vi "MQTT Data Stream - Decode HEADER.vi"(0 "TCP ref":refnum<k5>, 9 "timeout ms (1000)":i32, 11 "error in (no error)":errorcluster) -> (3 "RAW Data":string, 4 "TCP ref out":refnum<k5>, 6 "Fixed Header":T1, 15 "error out":errorcluster)   [LabVIEW 2019, in "KoRE-MQTT.lvlib"]
doc: "Decodes the MQTT fixed header byte.\n\n\nCopyright (c) 2025 KoRElibs.com\nSPDX-License-Identifier: EUPL-1.2\n\nThis VI is licensed under the European Union Public License (EUPL) Version 1.2. You may use this VI unmodified in proprietary works. If you distribute a modified version of this file, the modified file must be released under the EUPL-1.2. Full license: https://joinup.ec.europa.eu/asset/eupl/eupl/1.2/"
uses:
  KoRE-MQTT.lvlib
  TypeDefs/MQTT Packet - Fixed Header.ctl
  TypeDefs/MQTT Packet - Type.ctl
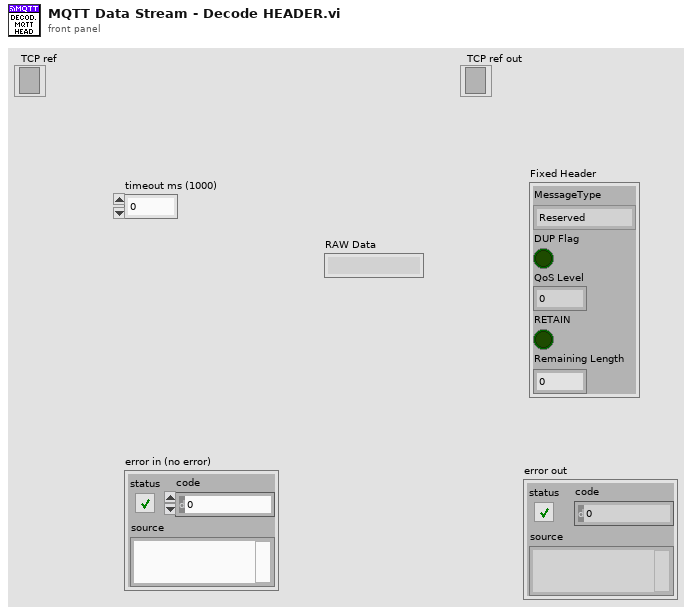
[diagram p1: front panel]
types:
  T1 = typedef "KoRE-MQTT.lvlib/MQTT Packet - Fixed Header.ctl" = cluster{"MessageType":T2, "DUP Flag":bool, "QoS Level":u8, "RETAIN":bool, "Remaining Length":u32}
  T2 = typedef "KoRE-MQTT.lvlib/MQTT Packet - Type.ctl" = enum32{"Reserved", "CONNECT", "CONNACK", "PUBLISH", "PUBACK", "PUBREC", "PUBREL", "PUBCOMP", "SUBSCRIBE", "SUBACK", "UNSUBSCRIBE", "UNSUBACK", "PINGREQ", "PINGRESP", "DISCONNECT", "AUTH"}
  T3 = enum16{"Standard", "Buffered", "CRLF", "Immediate"}
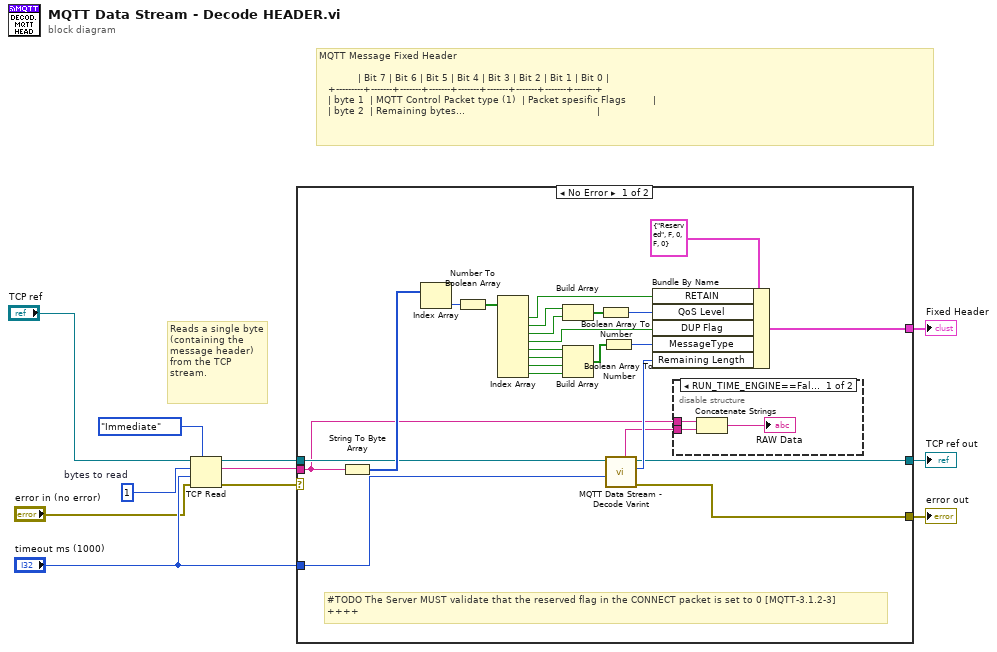
[diagram p0: block diagram]
diagram:
  w6 = 1  # bytes to read
  # "MQTT Message Fixed Header\n\n             | Bit 7 | Bit 6 | Bit 5 | Bit 4 | Bit 3 | Bit 2 | Bit 1 | Bit 0 |\n   +---------+-------+-------+-------+-------+-------+-------+-------+-------+\n   | byte 1  | MQTT Control Packet type (1)  | Packet spesific Flags         |\n   | byte 2  | Remaining bytes...                                            |"
  # "Reads a single byte (containing the message header) from the TCP stream."
  n1 = TCP Read(connection ID="TCP ref", bytes to read=w6, error in (no error)="error in (no error)", 7:T3."Immediate" ("mode (standard)"), 9:"timeout ms (1000)") -> (connection ID out=w7:refnum<k5>, data out=w9:string, error out=w4:errorcluster)
  n2 = case shown="No Error" w4 {
    selector: w4 -> [_ w40]
    tunnel: [w35 _] -> w11
    tunnel: "timeout ms (1000)" -> [w19 _]
    tunnel: w9 -> [w14 _]
    tunnel: w7 -> [w18 w39]
    tunnel: [w17 w40] -> w5
    tunnel: [w12 w39] -> w1
    frame No Error {
      # "#TODO The Server MUST validate that the reserved flag in the CONNECT packet is set to 0 [MQTT-3.1.2-3]\n++++"
      n3 = String To Byte Array(string=w14) -> (unsigned byte array=w31:u8[])
      n4 = Index Array(array=w31) -> (element=w20:u8)  [unwired: 1 in]
      n5 = Number To Boolean Array(number=w20) -> (Boolean array=w21:bool[])
      n6 = Index Array(array=w21) -> (element #1=w33:bool, element #2=w22:bool, element #3=w23:bool, element #4=w34:bool, element #5=w25:bool, element #6=w26:bool, element #7=w27:bool, element #8=w28:bool)  [unwired: 8 in]
      n7 = Build Array(w22, w23) -> (w24:bool[])
      n8 = Build Array(w25, w26, w27, w28) -> (w29:bool[])
      n9 = Boolean Array To Number(Boolean array=w24) -> (number=w15:u32)
      n10 = Boolean Array To Number(Boolean array=w29) -> (number=w16:u32)
      n11 = call "MQTT Data Stream - Decode Varint.vi"("timeout ms (1000)"=w19, "TCP Network Connection in"=w18) -> ("error out"=w17:errorcluster, "Numeric"=w32:u32, "TCP Network Connection out"=w12:refnum<k5>, "RAW data"=w13:string)  [unwired: 5 in, 1 out]
      n12 = Bundle By Name(cluster=T1 {"MessageType"=enum."Reserved", "DUP Flag"=FALSE, "QoS Level"=0, "RETAIN"=FALSE, "Remaining Length"=0} ("Fixed Header"), "RETAIN"=w33, "QoS Level"=w15, "DUP Flag"=w34, "MessageType"=w16, "Remaining Length"=w32) -> (w35:T1)
      n13 = disable-structure shown="RUN_TIME_ENGINE==False" {
        disable-tunnel: w14 -> [w38 _]
        disable-tunnel: w13 -> [w37 _]
        frame condition #0 (active) {
          n14 = Concatenate Strings(w38, w37) -> (→"RAW Data":string)
        }
        frame condition #1 {
        }
      }
    }
    frame Error {
    }
  }
  "Fixed Header" <- w11
  "error out" <- w5
  "TCP ref out" <- w1
